vi "simple_publisher.vi"() -> ()   [LabVIEW 2014]
panel:
  in  "停止":bool
  out "JSON字符串":string
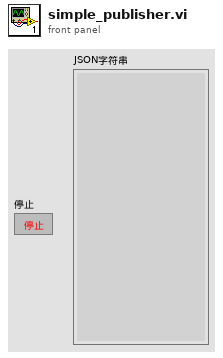
[diagram p1: front panel]
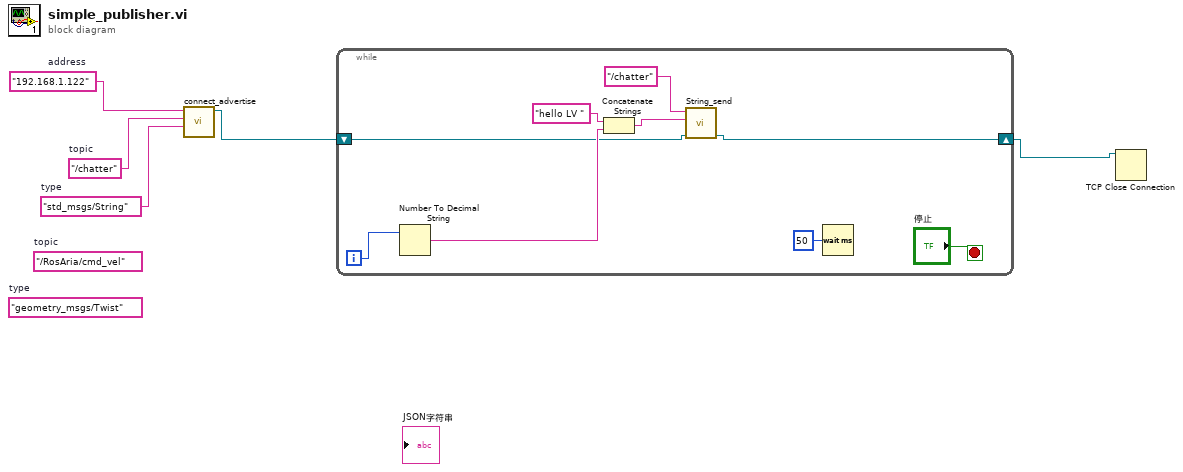
[diagram p0: block diagram]
diagram:
  w5 = "192.168.1.122"  # address
  w3 = "std_msgs/String"  # type
  w4 = "/chatter"  # topic
  (unwired) "geometry_msgs/Twist"  # type
  (unwired) "/RosAria/cmd_vel"  # topic
  n1 = call "connect_advertise.vi"("type"=w3, "topic"=w4, "address"=w5) -> ("连接ID输出"=w2:refnum<k5>)  [unwired: 7 in, 1 out]
  n2 = while {
    shift-right: [w6] -> w1
    shift-left: w2 -> [w7]
    i -> [w10]
    stop <- "停止" stop-if-true
    n3 = Number To Decimal String(number=w10) -> (decimal integer string=w9:string)  [unwired: 1 in]
    n4 = Concatenate Strings("hello LV " ("data"), w9) -> (w8:string)
    n5 = call "String_send.vi"("连接ID"=w7, "data"=w8, "topic"="/chatter") -> ("连接ID输出"=w6:refnum<k5>)  [unwired: 7 in, 1 out]
    n6 = Wait (ms)(milliseconds to wait=u32 50 ("等待时间（毫秒）")) -> ()  [unwired: 1 out]
  }
  n7 = TCP Close Connection(connection ID=w1) -> ()  [unwired: 2 in, 2 out]
